vi "Main.vi"(6 "Folder names":string[](array[string])=["StaARx#[PLC]StaATesterRxSignals", "StaATx#[PLC]StaATesterTxSignals"], 8 "error in":errorcluster, 9 "Sequence Context":refnum<k7>, 11 "TestExec In":refnum<class "TestExec.lvclass">) -> (0 "error out":errorcluster, 3 "TestExec Out":refnum<class "TestExec.lvclass">)   [LabVIEW 2025, in "TestExec.lvclass"]
uses:
  TestExec.lvclass
  TestExec.lvclass/TestExec.ctl
  Methods/Cylinder Display.vi
  <vilib>/addons/TestStand/_TSUtility.llb/TestStand - Get Property Value (Number {Signed 32-bit Integer}).vi
  OPC UA/Abstract.lvclass
panel:
  in  "Terminate":bool
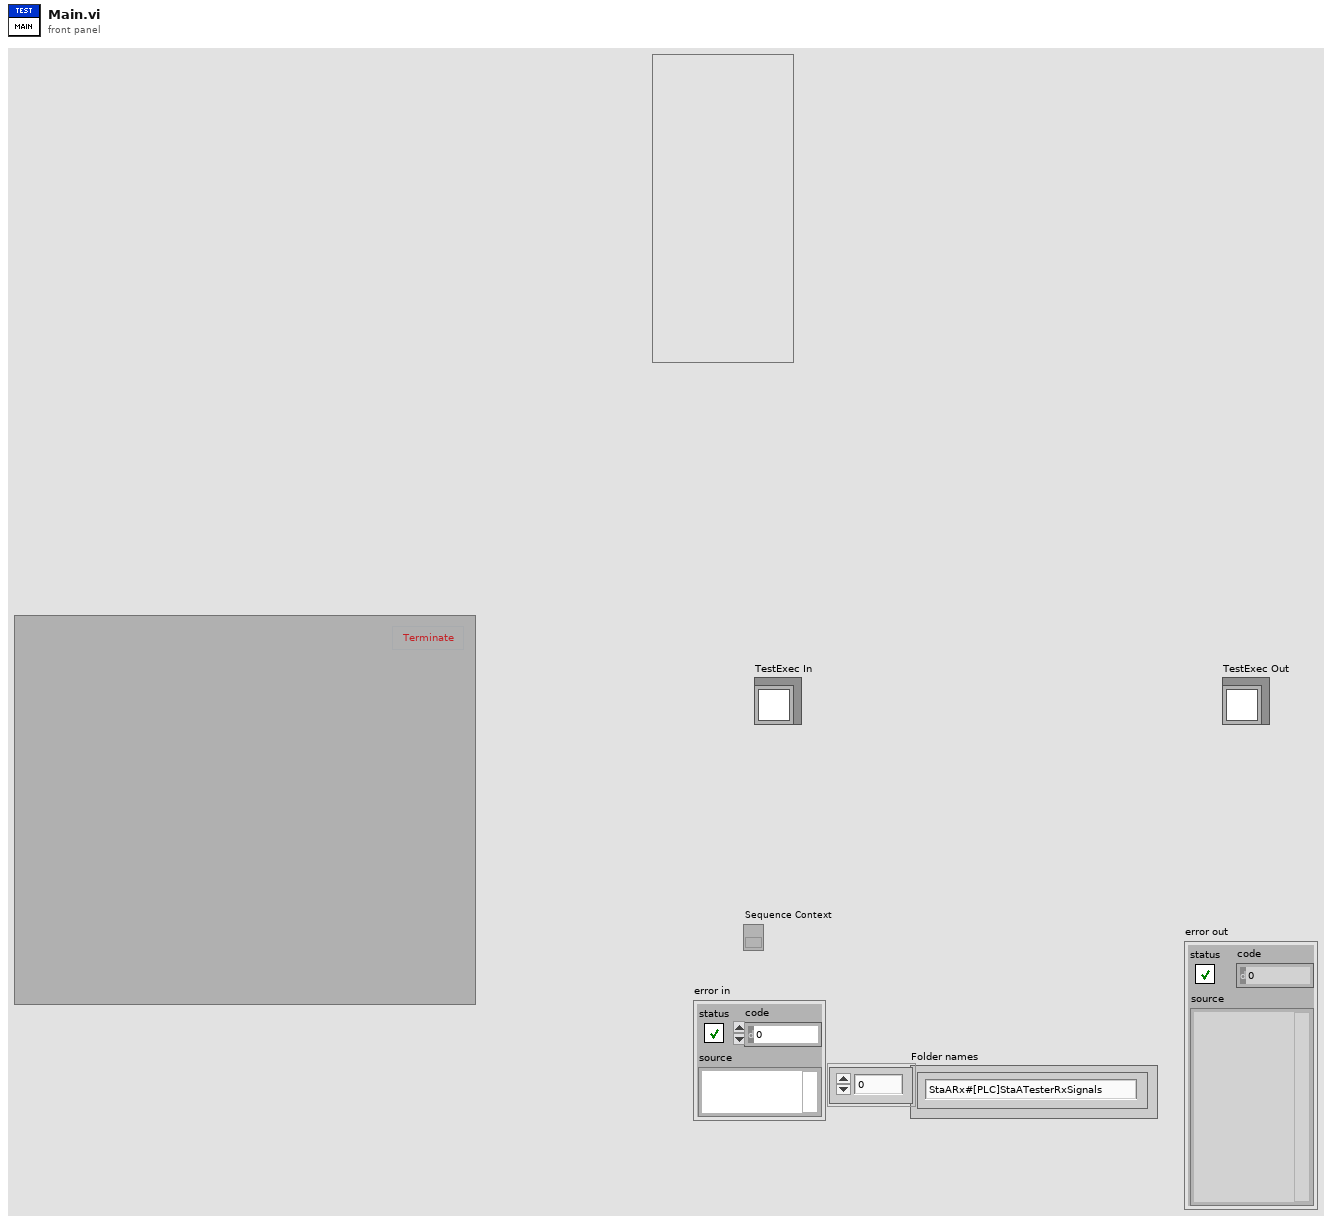
[diagram p1: front panel]
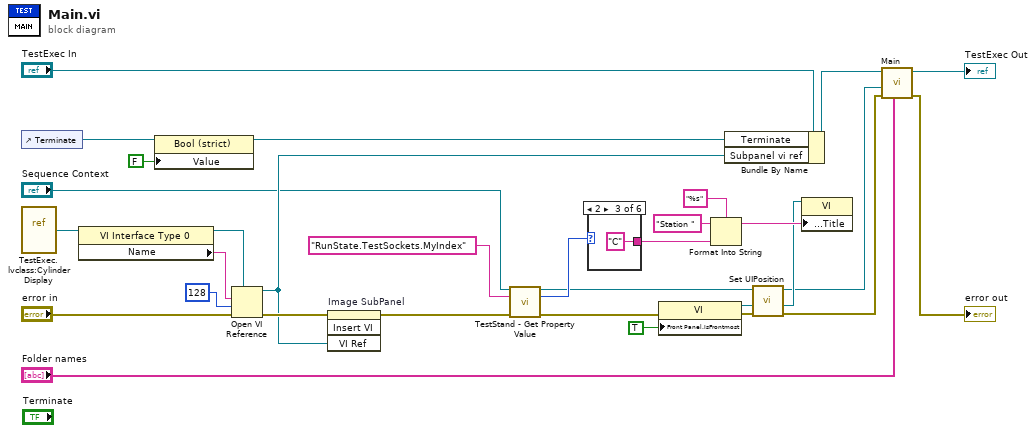
[diagram p0: block diagram]
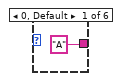
[diagram p2: hidden frame]
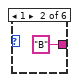
[diagram p3: hidden frame]
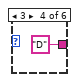
[diagram p4: hidden frame]
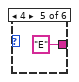
[diagram p5: hidden frame]
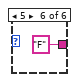
[diagram p6: hidden frame]
diagram:
  n1 = control-ref of="Terminate"() -> (w3:refnum<vi>)
  n2 = vi-ref "TestExec.lvclass:Cylinder Display.vi"() -> (w26:refnum<vi>)
  n3 = property on="Property Node" class="VI Interface Type 0"(reference=w26) -> (reference out=w28:refnum<vi>, "Name"=w27:string)  [unwired: 1 in, 1 out]
  n4 = property class="Bool (strict)"(reference=w3, "Value"=FALSE) -> (reference out=w1:refnum<vi>)  [unwired: 1 in, 1 out]
  n5 = Open VI Reference(type specifier VI Refnum (for type only)=w28, vi path=w27, options=128, error in (no error)="error in") -> (vi reference=w22:refnum<vi>, error out=w23:errorcluster)  [unwired: 2 in]
  n6 = invoke on="Image SubPanel" class="SubPnl" method="Insert VI"(error in=w23, "VI Ref"=w22) -> (error out=w4:errorcluster)  [unwired: 2 in, 3 out]
  n7 = call-poly <vilib>:"TestStand - Get Property Value.vi"("Sequence Context In"="Sequence Context", "Lookup String"="RunState.TestSockets.MyIndex", "error in (no error)"=w4) -> ("Sequence Context Out"=w8:refnum<k7>, "Value"=w11:i32, "error out"=w5:errorcluster)  [unwired: 10 in]
  n8 = case shown="2" w11 {
    tunnel: ["A" ("format string") "B" ("format string") "C" ("format string") "D" ("format string") "E" ("format string") "F" ("format string")] -> w16
    frame 0, Default {
    }
    frame 1 {
    }
    frame 2 {
    }
    frame 3 {
    }
    frame 4 {
    }
    frame 5 {
    }
  }
  n9 = property class="VI"(error in=w5, "Front Panel.IsFrontmost"=TRUE ("Front Panel Window:Is Frontmost")) -> (reference out=w17:refnum<vi>, error out=w18:errorcluster)  [unwired: 1 in]
  n10 = Format Into String(format string="%s", initial string="Station ", w16) -> (resulting string=w10:string)  [unwired: 1 in, 1 out]
  n11 = Bundle By Name(cluster="TestExec In", "Terminate"=w1, "Subpanel vi ref"=w22) -> (w20:refnum<class "TestExec.lvclass">)
  n12 = call "Set UIPosition.vi"("error in"=w18, "VI Ref"=w17, "Sequence Context In"=w8) -> ("error out"=w6:errorcluster, "reference out"=w9:refnum<vi>, "Sequence Context Out"=w7:refnum<k7>)  [unwired: 6 in]
  n13 = property class="VI"(reference=w9, "Front Panel.Title"=w10) -> ()  [unwired: 1 in, 2 out]
  n14 = call-parent "Main.vi"("Folder names"="Folder names", "error in"=w6, "Sequence Context"=w7, "OPC UA In"=w20) -> ("error out"=→"error out":errorcluster, "OPC UA Out"=→"TestExec Out":refnum<class "TestExec.lvclass">)  [unwired: 6 in]
